vi "Configure Tx Channel.vi"(8 "error in":errorcluster, 9 "labels settings for RT":T1[](array[typedef]) {"Label Timestamp Channel Data Reference" format="%.0x"; "Word Initial Raw Value" format="%032.0f"; "Label Disable/Trigger Channel Reference" format="%.0x"; "parameter driver data"."Tx parameter refs" format="%.0x"; "SDI" format="%02b"; "label" format="%.0o"}, 10 "channel number in":u8, 11 "board handle in":u8) -> (0 "error out":errorcluster, 1 "acyclic frame ids out":u32[](array[numeric]), 2 "channel number out":u8, 3 "board handle out":u8, 4 "Transfer ID map":map{u32, u32}(c390))   [LabVIEW 2020, in "AIM ARINC 429 Hardware API.lvlib"]
doc: "Configures all of the labels for a specified channel to be received."
uses:
  AIM ARINC 429 Hardware API.lvlib
  Shared/RT Label Settings.ctl
  Shared/Label.ctl
  Shared/RT Parameters.ctl
  Shared/Parameter Definition.ctl
  <vilib>/NI/NI VeriStand Encoding and Decoding/Encoding.ctl
  <vilib>/NI VeriStand/Custom Device API/Custom Device Item Ref.ctl
  Shared/Transfer Type.ctl
  <vilib>/NI VeriStand/Custom Device API/Data Reference.ctl
  <instrlib>/AIM GmbH/_ARINC-429/subvi/Error Converter (ErrCode or Status).vi
  <instrlib>/AIM GmbH/_ARINC-429/subvi/Get Library Path.vi
  <instrlib>/AIM GmbH/_ARINC-429/VIs/Library/Api429Lib Error Desc Get.vi
  <instrlib>/AIM GmbH/_ARINC-429/subvi/Get Error Number Offset.vi
  <vilib>/Utility/error.llb/Error Cluster From Error Code.vi
  <instrlib>/AIM GmbH/_ARINC-429/AIM429LV.lvlib
  <vilib>/NI/NI VeriStand Encoding and Decoding/Encoding and Decoding.lvlib
  <vilib>/NI VeriStand/Custom Device API/Custom Device API.lvlib
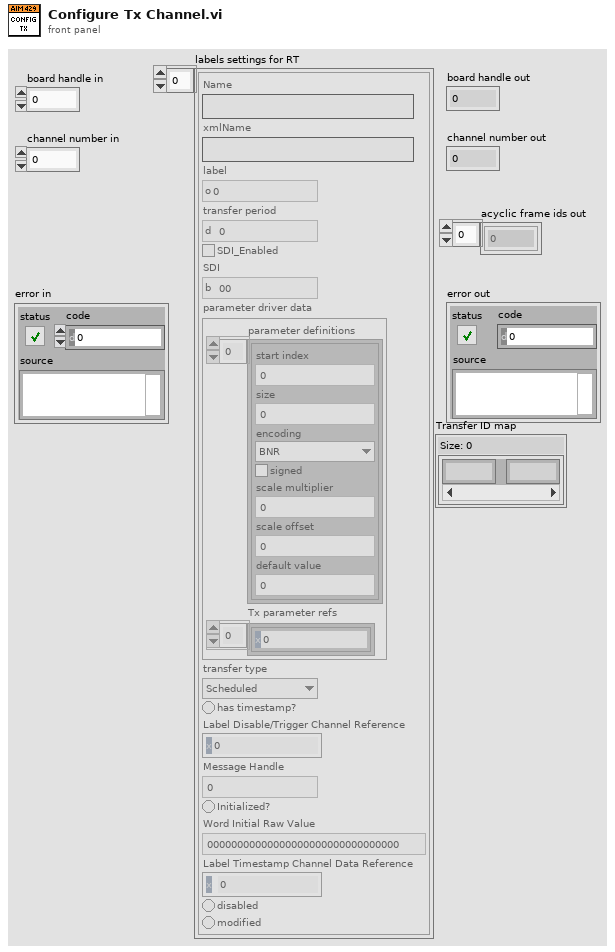
[diagram p1: front panel]
types:
  T1 = typedef "RT Label Settings.ctl" = cluster{"Name":string, "xmlName":string, "label":T2, "transfer period":u32, "SDI_Enabled":bool, "SDI":u8, "parameter driver data":T3, "transfer type":T7, "has timestamp?":bool, "Label Disable/Trigger Channel Reference":T6, "Message Handle":u64, "Initialized?":bool, "Word Initial Raw Value":u32, "Label Timestamp Channel Data Reference":T8, "disabled":bool, "modified":bool}
  T2 = typedef "Label.ctl" = u8
  T3 = typedef "RT Parameters.ctl" = cluster{"parameter definitions":T4[], "Tx parameter refs":T6[]}
  T4 = typedef "Parameter Definition.ctl" = cluster{"start index":i32, "size":i32, "encoding":T5, "signed":bool, "scale multiplier":dbl, "scale offset":dbl, "default value":dbl}
  T5 = typedef "Encoding and Decoding.lvlib/Encoding.ctl" = enum16{"BNR", "BCD", "Discrete"}
  T6 = typedef "Custom Device API.lvlib/Custom Device Item Ref.ctl" = u64
  T7 = typedef "Transfer Type.ctl" = enum16{"Scheduled", "Acyclic", "Block", "Strobe"}
  T8 = typedef "Custom Device API.lvlib/Data Reference.ctl" = i32
  T9 = cluster{"xfer_id":u32, "xfer_type":u32, "err_type":u32, "xfer_gap":u16, "ir_index":u16, "buf_size":u16, "xfer_ir":u8}
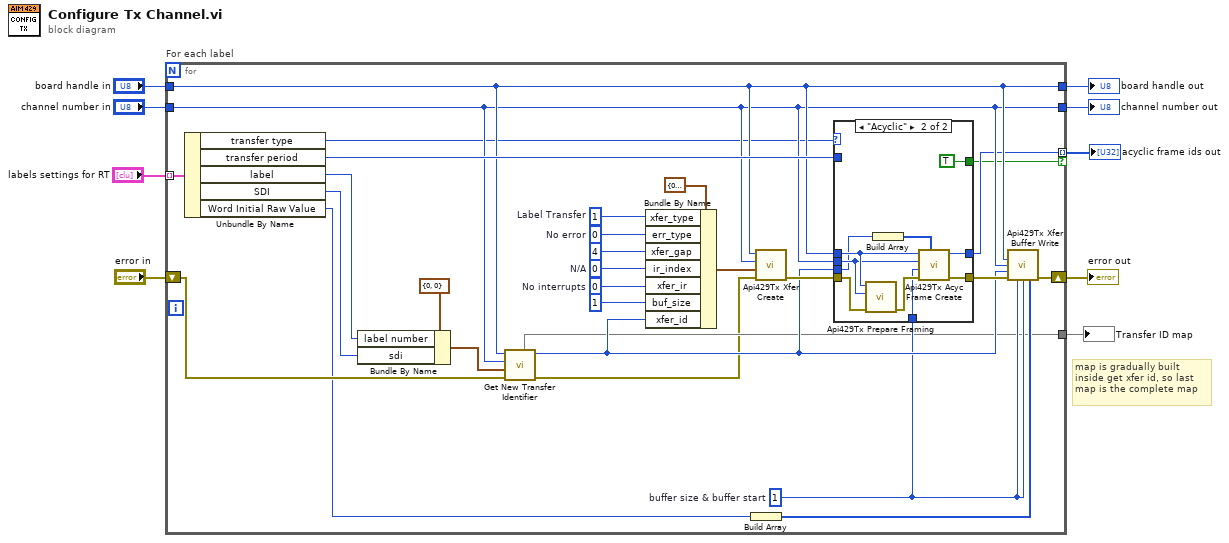
[diagram p0: block diagram]
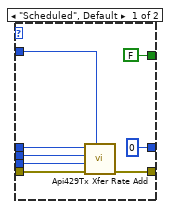
[diagram p2: hidden frame]
diagram:
  # "map is gradually built\ninside get xfer id, so last\nmap is the complete map"
  n1 = for "For each label" {
    tunnel: "channel number in" -> [w27]
    shift-right: [w24] -> w7
    shift-left: "error in" -> [w38]
    tunnel: "labels settings for RT" -> [w31] mode=indexing
    tunnel: [w27] -> w5
    tunnel: "board handle in" -> [w28]
    tunnel: [w28] -> w3
    tunnel: [w18] -> w2 mode=indexing if=w17
    tunnel: [w11] -> w1
    w19 = u16 1  # buffer size & buffer start
    w32 = u8 0  # No interrupts
    w34 = u16 0  # N/A
    w36 = u32 0  # No error
    w37 = u32 1  # Label Transfer
    n2 = Unbundle By Name(w31) -> ("transfer type"=w20:T7, "transfer period"=w30:u32, "label"=w14:T2, "SDI"=w13:u8, "Word Initial Raw Value"=w16:u32)
    n3 = Bundle By Name(cluster=cluster{"label number":T2, "sdi":u8} {"label number"=0, "sdi"=0} ("label information"), "label number"=w14, "sdi"=w13) -> (w12:cluster{"label number":T2, "sdi":u8})
    n4 = call "Get New Transfer Identifier.vi"("error in"=w38, "label information"=w12, "channel number in"=w27, "board number in"=w28) -> ("error out"=w10:errorcluster, "Transfer ID out"=w23:u32, "Transfer ID map"=w11:map{u32, u32})  [unwired: 4 in, 1 out]
    n5 = Bundle By Name(cluster=T9 {"xfer_id"=0, "xfer_type"=1, "err_type"=0, "xfer_gap"=0, "ir_index"=0, "buf_size"=0, "xfer_ir"=0} ("px_Xfer"), "xfer_type"=w37, "err_type"=w36, "xfer_gap"=u16 4 ("transfer gap in bits"), "ir_index"=w34, "xfer_ir"=w32, "buf_size"=u16 1 ("buffer size"), "xfer_id"=w23) -> (w22:T9)
    n6 = Build Array(w16) -> (w29:u32[])
    n7 = call <instrlib>:"Api429Tx Xfer Create.vi"("error in (no error)"=w10, "px_Xfer"=w22, "b_Chn"=w27, "board_handle"=w28) -> ("error out"=w26:errorcluster)  [unwired: 6 in, 1 out]
    n8 = case shown="\"Acyclic\"" w20 {
      tunnel: w30 -> [w46 _]
      tunnel: w28 -> [w45 w53]
      tunnel: w27 -> [w44 w52]
      tunnel: w26 -> [w43 w54]
      tunnel: [w42 w56] -> w25
      tunnel: w23 -> [w41 w50]
      tunnel: w19 -> [_ w51]
      tunnel: [u32 0 ("pulFrameId") w48] -> w18
      tunnel: [FALSE TRUE] -> w17
      frame "Scheduled", Default {
        n9 = call <instrlib>:"Api429Tx Xfer Rate Add.vi"("ulRateInMs"=w46, "error in (no error)"=w43, "ulXferId"=w41, "ucChannel"=w44, "board_handle"=w45) -> ("error out"=w42:errorcluster)  [unwired: 6 in]
      }
      frame "Acyclic" {
        n10 = call <instrlib>:"Api429Tx Prepare Framing.vi"("error in (no error)"=w54, "channel"=w52, "board_handle"=w53) -> ("error out"=w55:errorcluster)  [unwired: 8 in]
        n11 = Build Array(w50) -> (w49:u32[])
        n12 = call <instrlib>:"Api429Tx Acyc Frame Create.vi"("pulXfers"=w49, "error in (no error)"=w55, "ulXferCnt"=w51, "ucChannel"=w52, "board_handle"=w53) -> ("error out"=w56:errorcluster, "pulFrameId"=w48:u32)  [unwired: 5 in]
      }
    }
    n13 = call <instrlib>:"Api429Tx Xfer Buffer Write.vi"("board_handle"=w28, "b_Chn"=w27, "ul_XferId"=w23, "error in (no error)"=w25, "w_BufStart"=w19, "w_BufSize"=w19, "pl_LData"=w29) -> ("error out"=w24:errorcluster)  [unwired: 8 in]
  }
  "board handle out" <- w3
  "channel number out" <- w5
  "error out" <- w7
  "acyclic frame ids out" <- w2
  "Transfer ID map" <- w1
